vi "VIH - CHM Project - Get Project File Paths.vi"(8 "error in":errorcluster, 11 "Project Tree":T3) -> (0 "error out":errorcluster, 1 "Project Files":T2, 3 "dup Project Tree":T3)   [LabVIEW 2014]
doc: "::: VI Helpeks :::\nCopyright (c) 2000-2026 Konstantin Shifershteyn. All rights reserved."
uses:
  _VIH Project Manager.llb/VIH Project Tree Typedef - Tree Refnum.ctl
  _VIH HelpGen - Palette.llb/VIH HelpGen Typedef - Palette - Item Type Enum.ctl
panel:
  # "VI Helpeks\nCopyright (c) 2012-2026 Konstantin Shifershteyn"
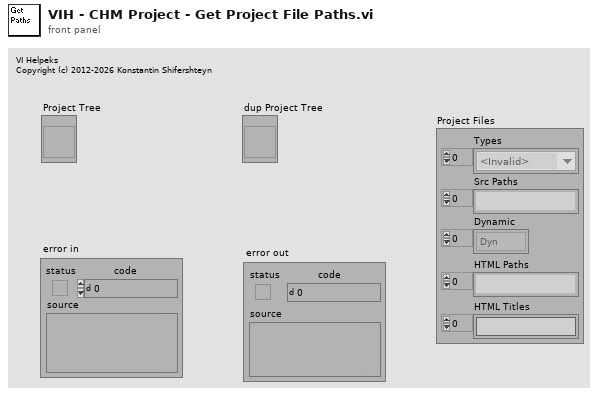
[diagram p1: front panel]
types:
  T1 = typedef "VIH HelpGen Typedef - Palette - Item Type Enum.ctl" = enum32{"<Invalid>", "<unknown>", "VI", "Menu", "LV Func", "Express VI", "Poly VI", "CTL", "HTML"}
  T2 = cluster{"Types":T1[], "Src Paths":path[], "Dynamic":enum16{"Dyn", "Stat", "Both"}[], "HTML Paths":path[], "HTML Titles":string[]}
  T3 = typedef "VIH Project Tree Typedef - Tree Refnum.ctl" = refnum<vi>
  T4 = cluster{"Types":T1[], "Paths":path[], "Dynamic":enum16{"Dyn", "Stat", "Both"}[], "Can be built":bool[], "DynFileNotFound":bool[]}
  T5 = typedef "VIH HelpGen Typedef - Cluster - File Rule.ctl" = cluster{"OutName":string, "BuildHelp":T6, "Source Paths":T7, "Target Paths":T8, "DscrMode":T9, "Description":string, "Control Rules":T10[], "Flags":T12, "Ctl_DscrMode":T9, "Ctl_ClustMembers":T6, "Ctl_EnumValues":T6, "MenuItemIcons":T6, "%Comments":string, "DetailsMode":T9, "DetailsText":string, "ProductInfoMode":T6, "ProductInfoText":string}
  T6 = typedef "VIH HelpGen Typedef - Enum - Default,Enable,Disable.ctl" = enum16{"Default", "Enable", "Disable"}
  T7 = typedef "VIH HelpGen Typedef - Cluster - File Rule - Source Paths.ctl" = cluster{"CSS Files":path[], "JS Files":path[], "Html Template":path}
  T8 = typedef "VIH HelpGen Typedef - Cluster - File Rule - Target Paths.ctl" = cluster{"HTML Dir":path, "Image Dir":path, "CSS Dir":path, "JS Dir":path}
  T9 = typedef "VIH HelpGen Typedef - Enum - Description Mode.ctl" = enum16{"Default", "Description", "Description1", "Description2", "Custom", "None"}
  T10 = typedef "VIH HelpGen Typedef - Cluster - Control Rule.ctl" = cluster{"CtrlID":string, "CustomRule":bool, "DscrMode":T9, "Description":string, "ClusterMembers":T6, "EnumValues":T6, "EnumValDscr":T11[], "CustomName":string}
  T11 = typedef "VIH HelpGen Typedef - Cluster - Enum Value Info.ctl" = cluster{"Value":ext, "String":string, "Description":string}
  T12 = typedef "VIH HelpGen Typedef - Cluster - Group Rule - Flags.ctl" = cluster{"Override CSS Files":bool, "Override JS Files":bool, "Override Ctl Rules":bool}
  T13 = cluster{T1[], path[], enum16{"Dyn", "Stat", "Both"}[], path[], string[]}
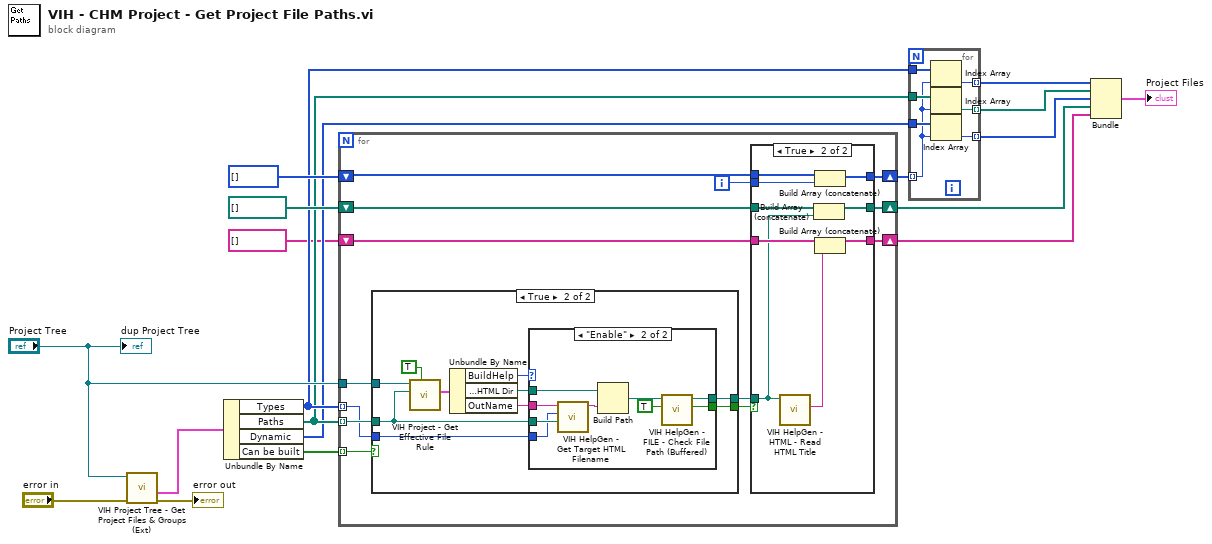
[diagram p0: block diagram]
diagram:
  n1 = call "VIH Project Tree - Get Project Files & Groups (Ext).vi"("error in"="error in", "Project Tree"="Project Tree") -> ("error out"=→"error out":errorcluster, "Project Files"=w13:T4)  [unwired: 6 in, 2 out]
  n2 = Unbundle By Name(w13) -> ("Types"=w12:T1[], "Paths"=w11:path[], "Dynamic"=w10:enum16{"Dyn", "Stat", "Both"}[], "Can be built"=w9:bool[])
  n3 = for {
    tunnel: "Project Tree" -> [w31]
    tunnel: w11 -> [w30] mode=indexing
    tunnel: w12 -> [w29] mode=indexing
    tunnel: w9 -> [w28] mode=indexing
    shift-right: [w24] -> w3
    shift-left: path[] [] -> [w25]
    shift-right: [w21] -> w5
    shift-left: i32[] [] -> [w22]
    shift-right: [w19] -> w1
    shift-left: string[] [] -> [w20]
    i -> [w23]
    n4 = case shown="True" w28 {
      tunnel: w31 -> [_ w49]
      tunnel: w30 -> [_ w48]
      tunnel: w29 -> [_ w47]
      tunnel: [_ w46] -> w27
      tunnel: [_ w45] -> w26
      frame False {
      }
      frame True {
        n5 = call "VIH Project - Get Effective File Rule.vi"("Ignore Control Rules (F)"=TRUE, "File Path"=w48, "Project Tree"=w49) -> ("Effective File Rule"=w53:T5)  [unwired: 5 in, 3 out]
        n6 = Unbundle By Name(w53) -> ("BuildHelp"=w44:T6, "Target Paths.HTML Dir"=w50:path, "OutName"=w51:string)
        n7 = case shown="\"Enable\"" w44 {
          tunnel: w51 -> [_ w60]
          tunnel: w50 -> [_ w59]
          tunnel: w48 -> [_ w57]
          tunnel: w47 -> [_ w56]
          tunnel: [_ w55] -> w46
          tunnel: [_ w54] -> w45
          frame Default {
          }
          frame "Enable" {
            n8 = call "VIH HelpGen - Get Target HTML Filename.vi"("Item File Path"=w57, "Item Type"=w56, "HTML Filename in"=w60) -> ("HTML Fileame out"=w58:string)  [unwired: 7 in, 1 out]
            n9 = Build Path(base path=w59, name or relative path=w58) -> (appended path=w61:path)
            n10 = call "VIH HelpGen - FILE - Check File Path (Buffered).vi"("Force Update (T)"=TRUE, "File Path"=w61) -> ("Good path"=w55:bool, "dup File Path"=w54:path)  [unwired: 8 in]
          }
        }
      }
    }
    n11 = case shown="True" w27 {
      tunnel: w26 -> [_ w36]
      tunnel: w25 -> [w34 w43]
      tunnel: [w34 w42] -> w24
      tunnel: w23 -> [_ w41]
      tunnel: w22 -> [w33 w40]
      tunnel: [w33 w39] -> w21
      tunnel: w20 -> [w32 w38]
      tunnel: [w32 w37] -> w19
      frame False {
      }
      frame True {
        n12 = call "VIH HelpGen - HTML - Read HTML Title.vi"("HTML File Path"=w36) -> ("Title"=w35:string)  [unwired: 8 in, 2 out]
        n13 = Build Array (concatenate)(w43, w36) -> (w42:path[])
        n14 = Build Array (concatenate)(w40, w41) -> (w39:i32[])
        n15 = Build Array (concatenate)(w38, w35) -> (w37:string[])
      }
    }
  }
  n16 = for {
    tunnel: w12 -> [w69]
    tunnel: w11 -> [w68]
    tunnel: w10 -> [w67]
    tunnel: [w66] -> w8 mode=indexing
    tunnel: [w65] -> w6 mode=indexing
    tunnel: w5 -> [w64] mode=indexing
    tunnel: [w63] -> w4 mode=indexing
    n17 = Index Array(array=w69, index=w64) -> (element=w66:T1)
    n18 = Index Array(array=w68, index=w64) -> (element=w65:path)
    n19 = Index Array(array=w67, index=w64) -> (element=w63:enum16{"Dyn", "Stat", "Both"})
  }
  n20 = Bundle(w8, w6, w4, w3, w1) -> (→"Project Files":T13)  [unwired: 1 in]
  "dup Project Tree" <- "Project Tree"
